vi "CSM - Debug Console 2.vi"() -> ()   [LabVIEW 2017, in "DebugConsole.lvlib"]
doc: "New version of the CSM Debug Console, you can use this tool:\n1. Select an existing CSM instance, open the front panel and block diagram.\n2. Scan the API interfaces of existing CSM instances.\n3. Select an API interface, call synchronously or asynchronously, view the return value.\n4. View the overall program's running log.\n5. Run Scripts."
uses:
  DebugConsole.lvlib
  _Support/Typedef/_CSM_List Module Scope.ctl
  _Support/Typedef/_CSM_GlobalLog_MSG.ctl
  _Support/Typedef/_CSM_Response Source Message.ctl
  _Support/Typedef/_CSM_GlobalLog_MSG_TYPE.ctl
  _BroadcastDef.ctl
  AdvanceAPI/CSM - Convert Error to Argument.vi
  _Support/GlobalEvent/GEvt-Generate with Rule Check.vi
  _Support/GlobalEvent/Cache-GEvt Refs.vi
  AdvanceAPI/CSM - Keywords.vi
  AdvanceAPI/CSM - Make String Arguments Safe.vi
  _Support/ChangeFlag/FlagInstance-GEvt Refs.vi
  _Support/ChangeFlag/ChangeFlag-Read.vi
  _csmHelper/API/Create From VI Reference.vi
  _csmHelper/API/Update lvcsm Section in VI Description.vi
  _csmHelper/API/Destroy.vi
  _csmlite/_PassAllowedMessage - MsgList.vi
  _Support/ChangeFlag/ChangeFlagDB.vi
  _Support/GlobalEvent/FGV-GlobalEventRef(lvlibp).vi
  _Support/GlobalEvent/FGV-GlobalEventQueues(lvlibp).vi
  _Support/GlobalEvent/GEvt-Valid Subscribers.vi
  _Support/GlobalEvent/LogFilter/LogFilter - Check.vi
  HistoryList.vi
  Script-Window.vi
  Module Information.vi
  _Support/GlobalEvent/LogFilter/LogFilter.lvclass
  Communicable State Machine.lvlib
  _csmHelper/API with lvcsm Support/CSM-Helper API with lvcsm Support.lvlib
  _csmHelper/CSM-Helper.lvclass
  _ui/csm-ui-support.lvlib
  _csmlite/_csmlite.lvlib
  _Shared/CSM Shared.lvlib
  _csmlite/_action.ctl
panel:
  in  "Scope":T1
  in  "Refresh CSMs Button":bool
  in  "CSM":string(combo)
  in  "Write lvcsm in Description":bool
  out "inlvlibp":bool
  in  "RetainWireValues":bool
  in  "Toolbar.Exit":bool
  in  "Toolbar.Open FP":bool
  in  "Toolbar.Open BD":bool
  in  "Refresh lvcsm Cache":bool
  in  "Console":T2(tab)
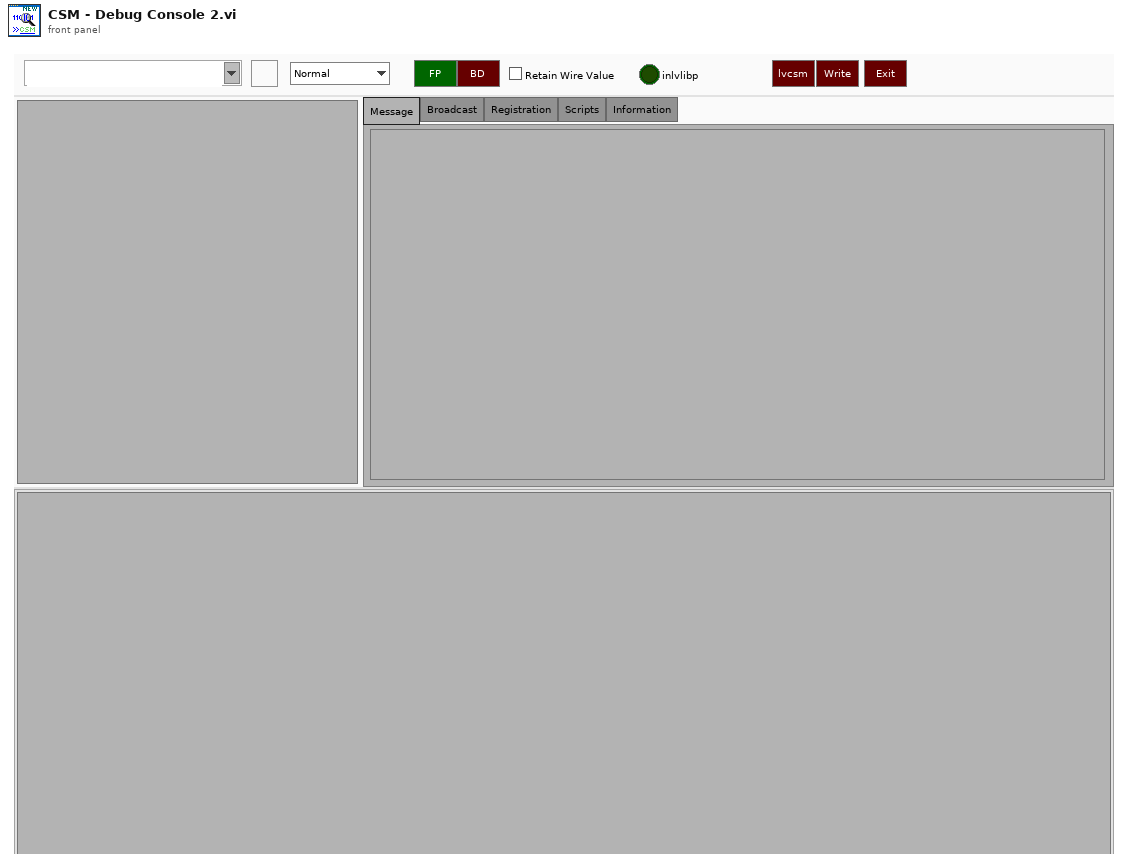
[diagram p1: front panel]
types:
  T1 = typedef "Communicable State Machine.lvlib/_CSM_List Module Scope.ctl" = enum16{"Normal", "System Only", "All"}
  T2 = enum32{"Message", "Broadcast", "Registration", "Scripts", "Information"}
  T3 = cluster{"Left":i32, "Right":i32, "Top":i32, "Bottom":i32}
  T4 = enum32{"Invalid", "Standard", "Closed", "Hidden", "Minimized", "Maximized"}
  T5 = enum32{"invalid app kind", "Development System", "Run Time System", "Student Edition", "Embedded LabVIEW", "Evaluation", "Custom"}
  T6 = typedef "DebugConsole.lvlib/_BroadcastDef.ctl" = enum16{"<no action>", "Macro: Exit", "CSM: Module List Changed", "CSM: Scripts Changed", "CSM: Registration Changed", "CSM: Module Selected", "CSM: Message Excuted", "CSM: Broadcast Excuted", "CSM: Registration Action Excuted", "UI: Try to Change Command"}
  T7 = typedef "_csmlite.lvlib/_action.ctl" = enum16{"Obtain", "Destroy", "Broadcast", "Post", "List"}
  T8 = cluster{"Shift":bool, "Ctrl":bool, "Alt":bool, "Cmd":bool, "Opt":bool}
  T9 = cluster{"Core":cluster{"Current VI Reference":refnum<vi>, "Close Panel on Exit?":bool}, "CSM Global Log Event":refnum<user-event>, "MessageList":string[], "Toobar.advance":refnum<vi>[], "ConsoleUI":refnum<vi>[]}
  T10 = cluster{"Current VI Reference":refnum<vi>, "Close Panel on Exit?":bool}
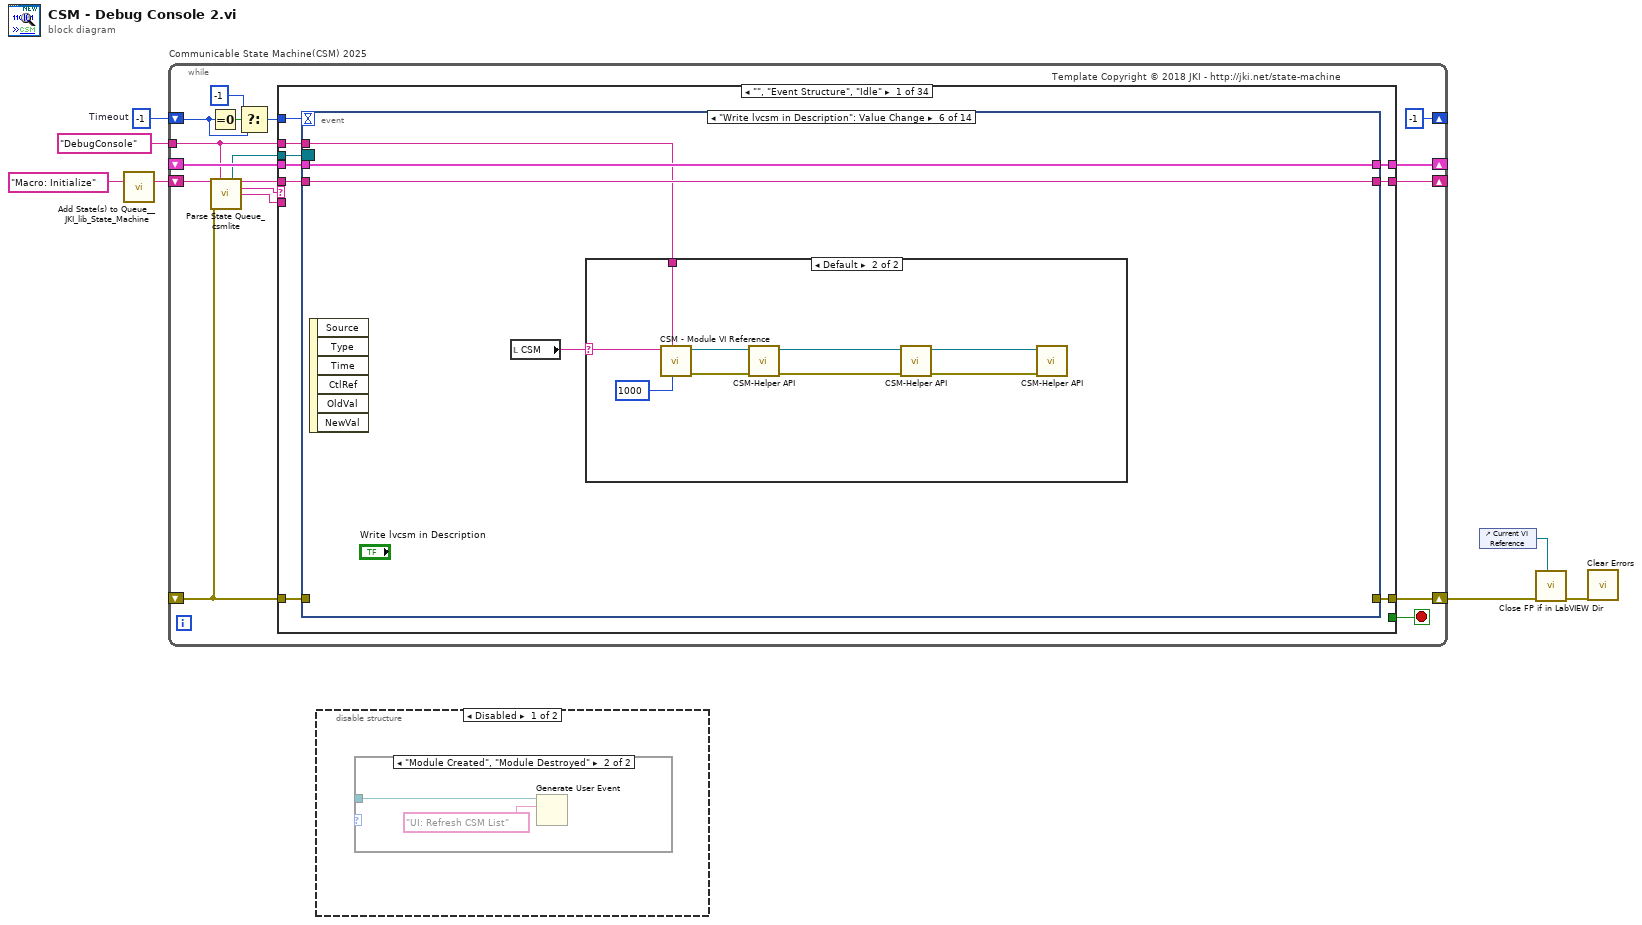
[diagram p0: block diagram]
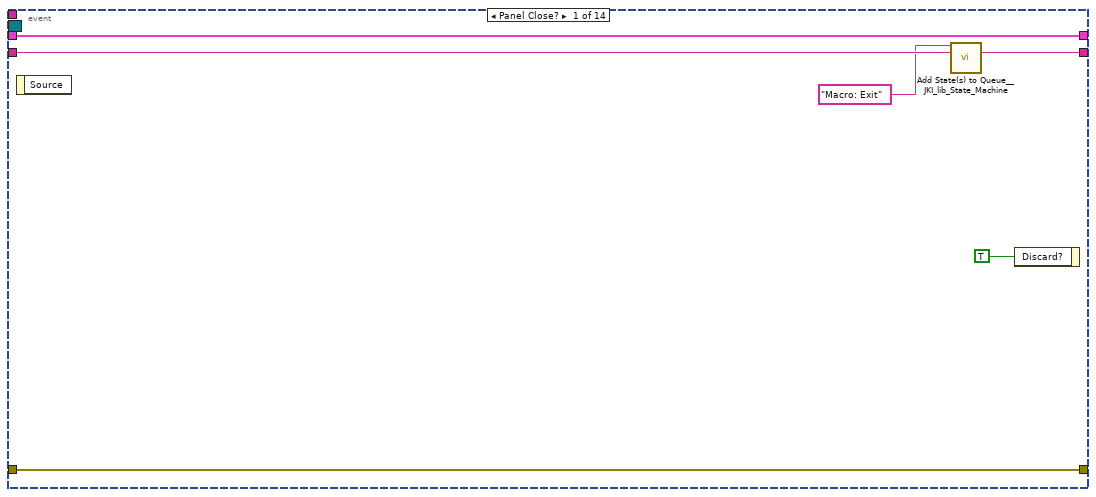
[diagram p4: hidden frame]
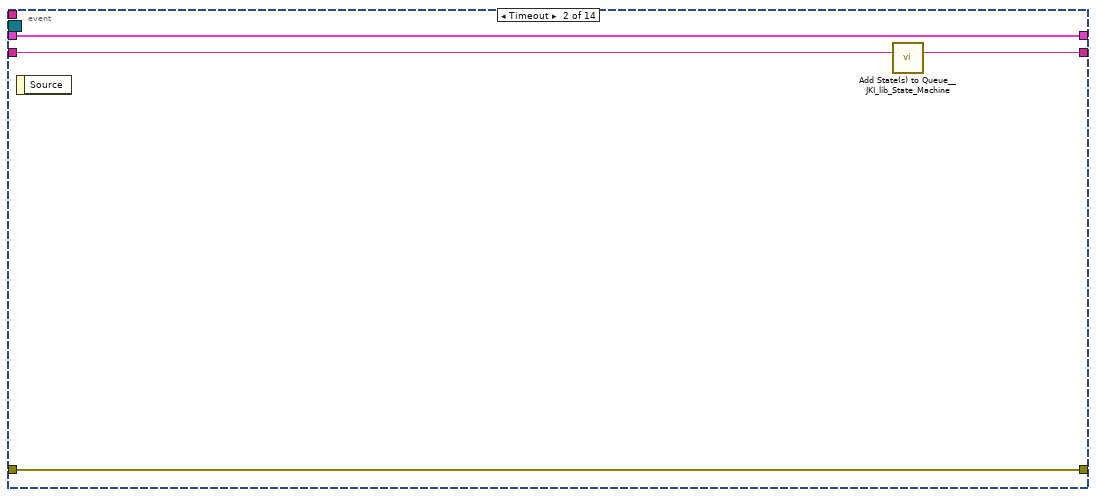
[diagram p5: hidden frame]
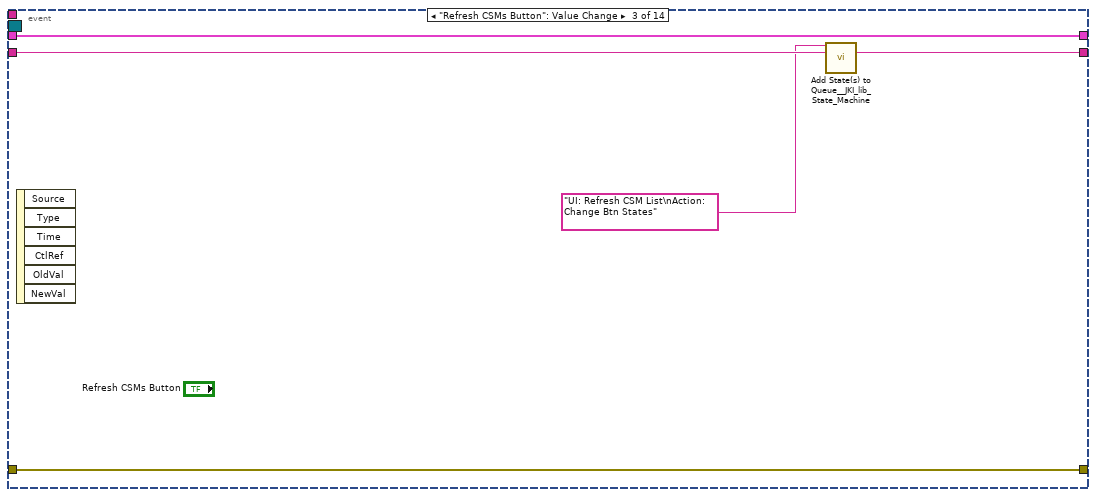
[diagram p6: hidden frame]
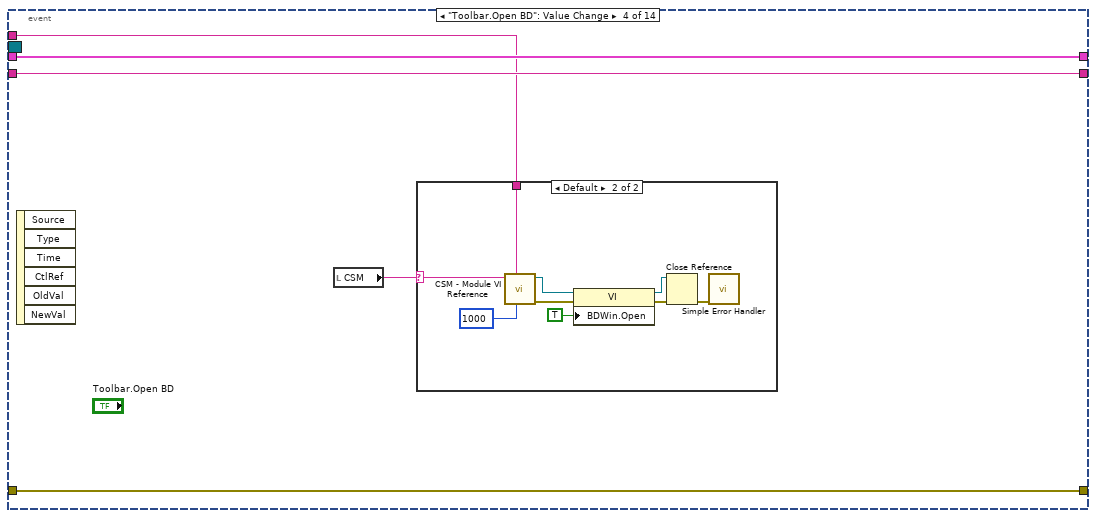
[diagram p7: hidden frame]
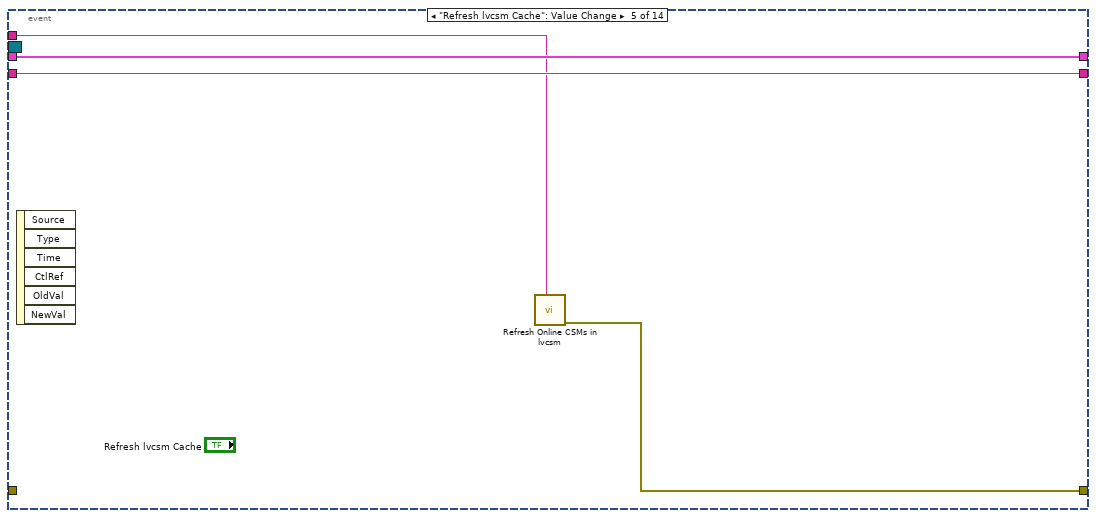
[diagram p9: hidden frame]
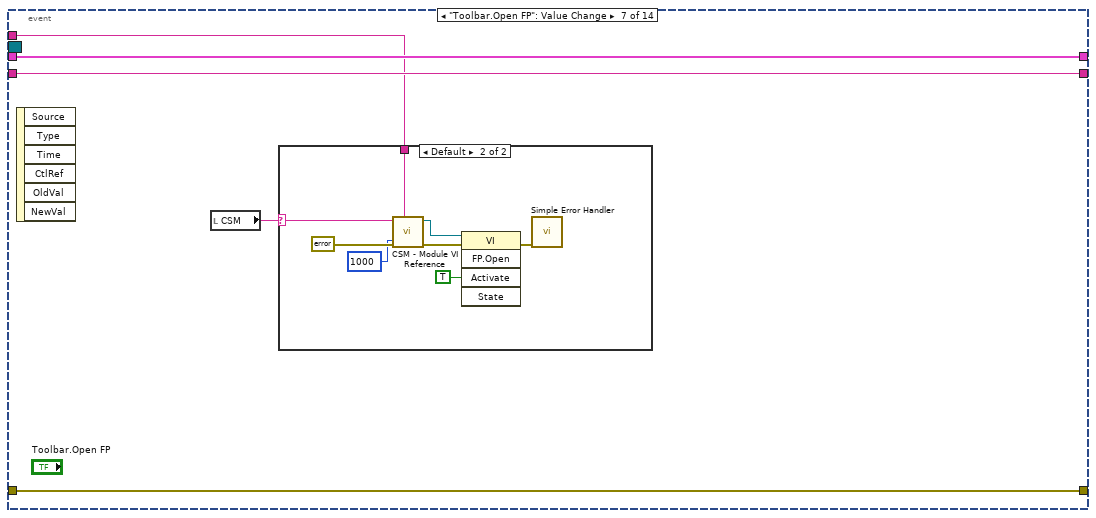
[diagram p11: hidden frame]
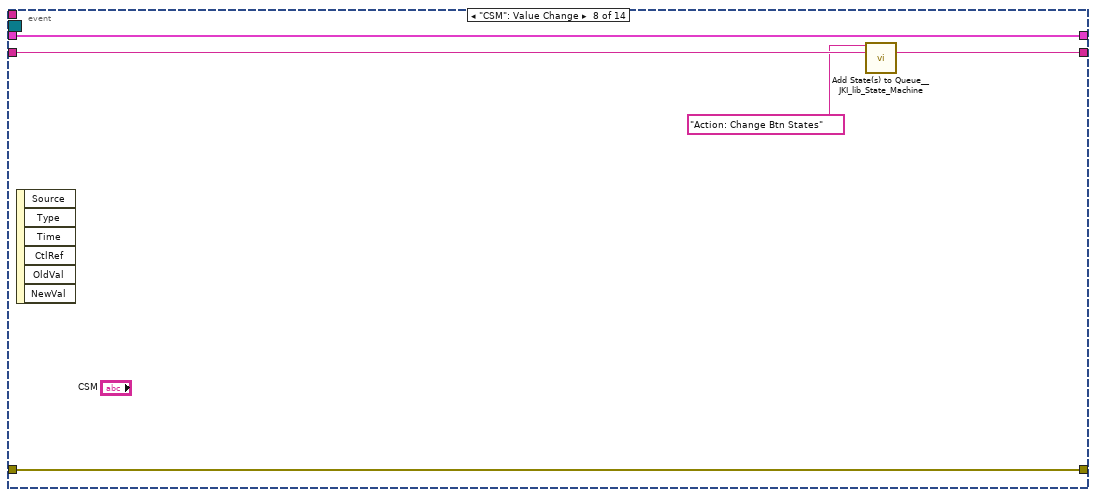
[diagram p13: hidden frame]
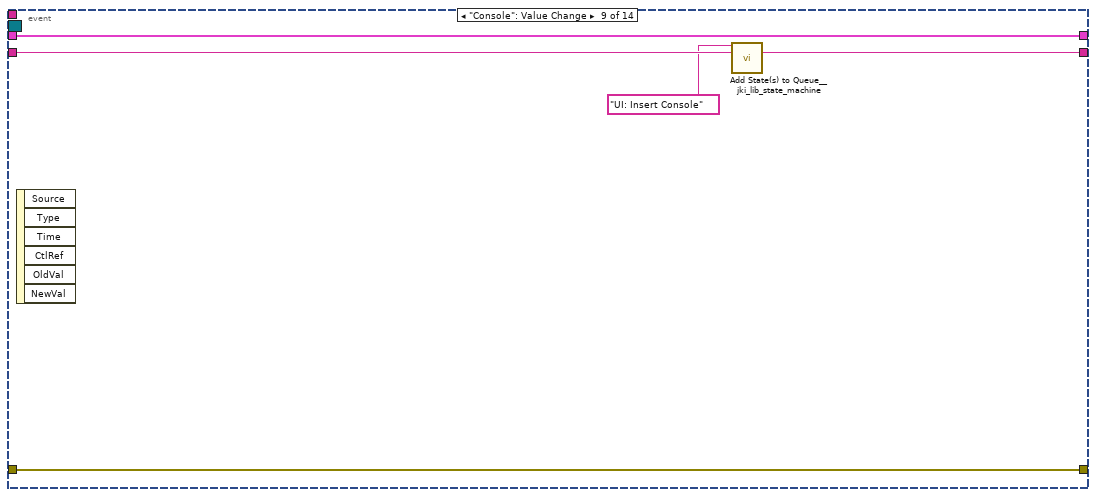
[diagram p14: hidden frame]
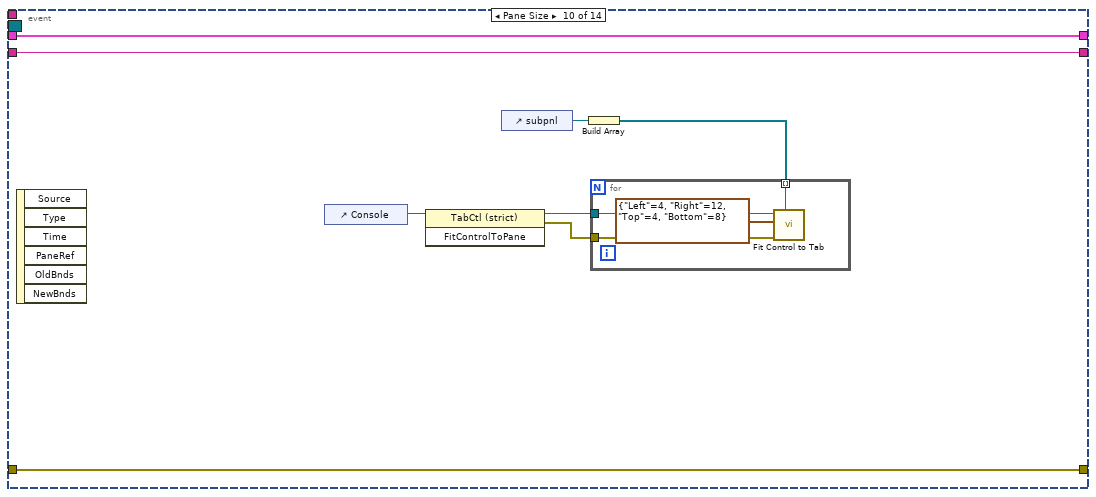
[diagram p15: hidden frame]
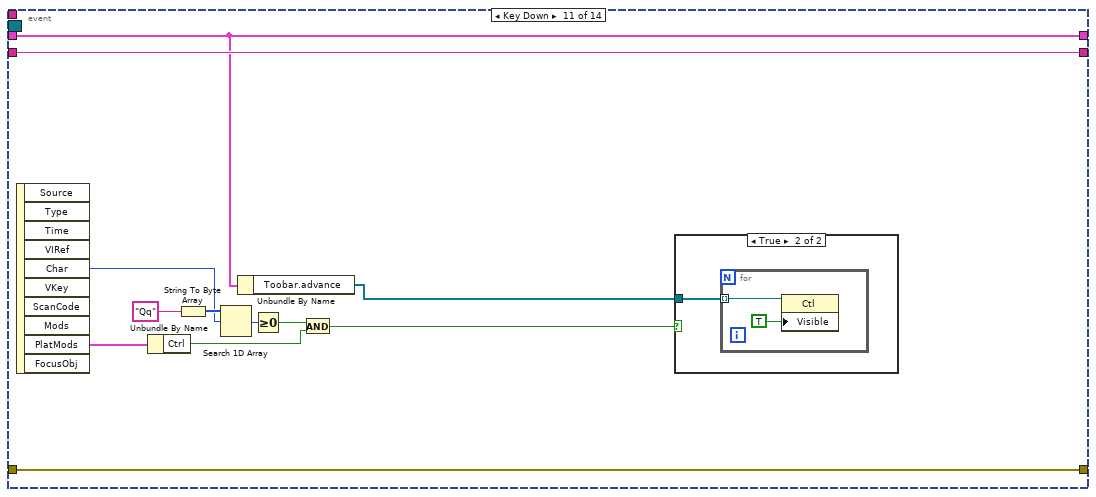
[diagram p16: hidden frame]
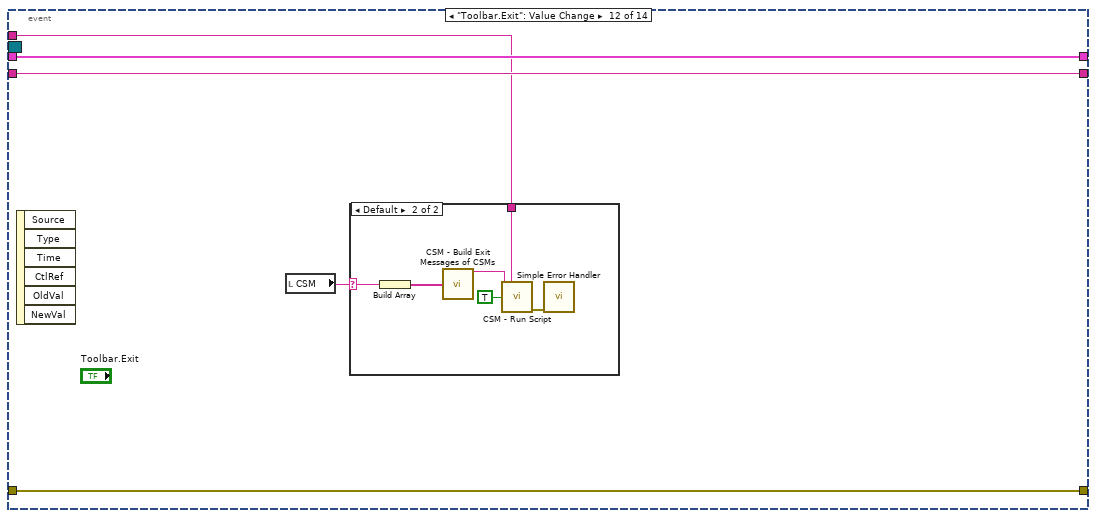
[diagram p18: hidden frame]
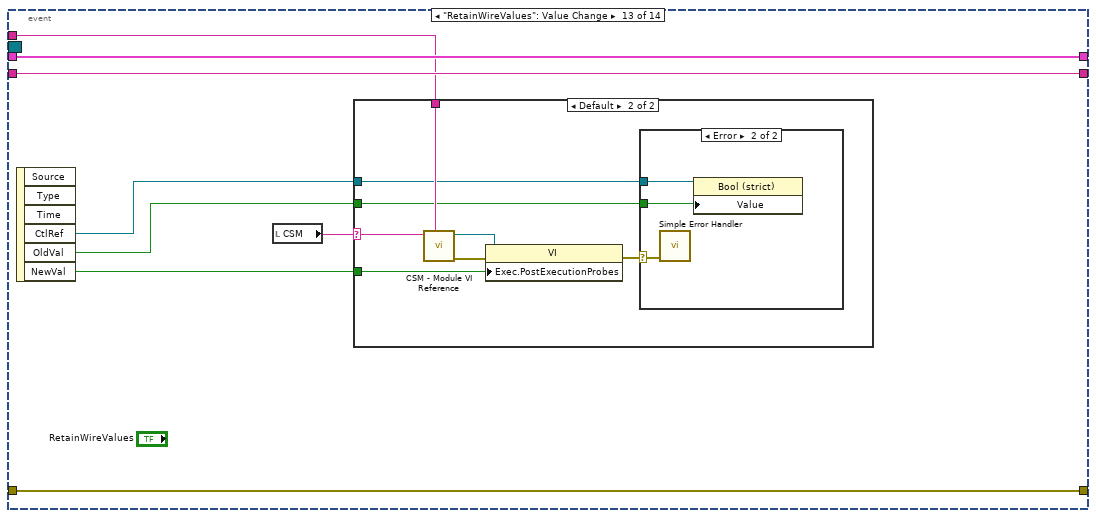
[diagram p20: hidden frame]
diagram:
  w5 = -1  # Timeout
  n1 = call <vilib>:"Add State(s) to Queue__JKI_lib_State_Machine.vi"("State(s) in (\"\")"="Macro: Initialize") -> ("States Out"=w6:string)  [unwired: 14 in]
  n2 = while "Communicable State Machine(CSM) 2025" {
    shift-right: [w17] -> _
    shift-left: _ -> [w16]
    shift-right: [w20] -> w2
    shift-left: _ -> [w15]
    shift-right: [w19] -> _
    shift-left: w6 -> [w21]
    tunnel: "DebugConsole" -> [w9]
    shift-right: [-1 ("Timeout")] -> _
    shift-left: w5 -> [w12]
    stop <- w18 stop-if-true
    # "Template Copyright © 2018 JKI - http://jki.net/state-machine"
    n3 = Equal To 0?(x=w12) -> (x = 0?=w14:bool)
    n4 = call "Parse State Queue_csmlite.vi"("State Queue"=w21, "Current Module(\"\" to generate an ID)"=w9, "Error In (no error)"=w15) -> ("Event Registration Refnum"=w8:refnum<event-registration>, "Remaining States"=w23:string, "Current State"=w24:string, "Arguments"=w22:string)  [unwired: 9 in]
    n5 = Select(t=-1 ("Timeout"), s=w14, f=w12) -> (s? t:f=w11:i32)
    n6 = case shown="\"\", \"Event Structure\", \"Idle\"" w24 {
      selector: w24 -> [_ _ w171 _ _ _ _ _ _ _ _ _ _ _ _ _ _ _ _ _ _ _ _ _ _ _ _ _ _ _ _ _ _ _]
      tunnel: w23 -> [w33 w170 w175 w194 w201 w206 w210 w219 w226 w229 w231 w241 w256 w260 w270 w280 w291 w368 w385 w405 w421 w428 w431 w436 w441 w452 w473 w479 w498 w503 w522 w541 w560 w579]
      tunnel: w22 -> [_ _ _ _ _ _ _ _ _ _ _ w237 _ _ _ w275 w285 _ w382 _ _ _ _ _ _ _ _ _ _ _ _ _ _ _]
      tunnel: w16 -> [w31 w167 w173 w187 w198 w204 w207 _ w225 w228 w230 w239 w251 w257 w267 w278 w287 w367 w384 w404 w420 w426 w430 w433 w438 w449 w470 w478 w497 w502 w521 w540 w559 w578]
      tunnel: [w30 w168 w177 w191 errorcluster {"status"=FALSE, "code"=0, "source"=""} ("error out") w203 w208 w216 w227 _ _ w240 w252 w258 w268 w276 w288 w369 w386 w406 w422 w429 w432 w434 w439 w450 w471 w480 w499 w504 w523 w542 w561 w580] -> w20
      tunnel: w15 -> [w29 w168 w176 w191 w197 w203 w208 w216 w227 _ _ w240 w253 w258 w268 w277 w289 w369 w386 w406 w422 w429 w432 w434 w439 w450 w471 w480 w499 w504 w523 w542 w561 w580]
      tunnel: [w32 w169 w174 w193 w200 w205 w209 w218 w226 w229 w231 w241 w255 w259 w269 w279 w290 w368 w385 w405 w421 w428 w431 w435 w440 w451 w472 w479 w498 w503 w522 w541 w560 w579] -> w19
      tunnel: [_ _ _ _ _ TRUE _ _ _ _ _ _ _ _ _ _ _ _ _ _ _ _ _ _ _ _ _ _ _ _ _ _ _ _] -> w18
      tunnel: [w28 w167 w173 w192 w198 w204 w207 w217 w222 w228 w230 w233 w251 w257 w267 w278 w287 w367 w384 w404 w420 w426 w430 w433 w438 w449 w470 w478 w497 w501 w520 w539 w558 w577] -> w17
      tunnel: w11 -> [w27 _ _ _ _ _ _ _ _ _ _ _ _ _ _ _ _ _ _ _ _ _ _ _ _ _ _ _ _ _ _ _ _ _]
      tunnel: w9 -> [w26 _ _ _ w195 _ _ _ _ _ _ _ _ _ _ _ _ _ _ w393 w409 _ _ _ _ w442 _ w476 w495 w500 w519 w538 w557 w576]
      tunnel: w8 -> [w25 _ _ _ _ _ _ _ _ _ _ _ _ _ _ _ _ _ _ _ _ _ _ _ _ _ _ _ _ _ _ _ _ _]
      frame "", "Event Structure", "Idle" {
        n7 = event shown="[5] \"Write lvcsm in Description\": Value Change" {
          selector: w25 -> [_ _ _ _ _ _ _ _ _ _ _ _ _ _]
          dyn-events: _ -> [_ _ _ _ _ _ _ _ _ _ _ _ _ _]
          timeout: w27 -> [_ _ _ _ _ _ _ _ _ _ _ _ _ _]
          tunnel: w33 -> [w39 w43 w46 w53 w66 w70 w84 w94 w99 w110 w126 w134 w148 w163]
          tunnel: [w38 w42 w45 w53 w66 w70 w84 w95 w100 w110 w126 w134 w148 w164] -> w32
          tunnel: w31 -> [w36 w40 w47 w52 w65 w69 w83 w96 w101 w108 w115 w133 w146 w165]
          tunnel: [w37 w41 w48 w50 w63 _ w81 w97 w102 w109 w125 w132 w147 w166] -> w30
          tunnel: w29 -> [w37 w41 w48 w50 _ _ w81 w97 w102 w109 w125 w132 w147 w166]
          tunnel: [w36 w40 w47 w52 w65 w69 w83 w96 w101 w108 w115 w133 w146 w165] -> w28
          tunnel: w26 -> [_ _ _ w49 w64 w67 w80 _ _ _ _ w130 w144 _]
          event Panel Close? {
            n8 = event-data() -> ()  [unwired: 1 in, 1 out]
            n9 = call <vilib>:"Add State(s) to Queue__JKI_lib_State_Machine.vi"("State(s) in Front (\"\")"="Macro: Exit", "State(s) in (\"\")"=w39) -> ("States Out"=w38:string)  [unwired: 13 in]
            n10 = event-data("Discard?"=TRUE) -> ()  [unwired: 1 in, 1 out]
          }
          event Timeout {
            n11 = event-data() -> ()  [unwired: 1 in, 1 out]
            n12 = call <vilib>:"Add State(s) to Queue__JKI_lib_State_Machine.vi"("State(s) in (\"\")"=w43) -> ("States Out"=w42:string)  [unwired: 14 in]
          }
          event "Refresh CSMs Button": Value Change {
            n13 = event-data() -> ()  [unwired: 1 in, 6 out]
            n14 = call <vilib>:"Add State(s) to Queue__JKI_lib_State_Machine.vi"("State(s) in Front (\"\")"="UI: Refresh CSM List\nAction: Change Btn States" ("State(s) in Front (\"\")"), "State(s) in (\"\")"=w46) -> ("States Out"=w45:string)  [unwired: 13 in]
          }
          event "Toolbar.Open BD": Value Change {
            n15 = event-data() -> ()  [unwired: 1 in, 6 out]
            n16 = local read "CSM"() -> (w51:string)
            n17 = case shown="Default" w51 {
              selector: w51 -> [_ w61]
              tunnel: w49 -> [_ w60]
              frame "" {
              }
              frame Default {
                n18 = call "CSM - Module VI Reference.vi"("Response Timeout (-2 Using Global Settings)"=1000 ("Response Timeout(5000 ms)"), "Current Module (\"\" to Generate an ID)"=w60, "CSM Name"=w61) -> ("error out"=w54:errorcluster, "CSM Module VIRef"=w59:refnum<vi>)  [unwired: 7 in]
                n19 = property class="VI"(reference=w59, error in=w54, "BDWin.Open"=TRUE ("Block Diagram Window:Open")) -> (reference out=w57:refnum<vi>, error out=w56:errorcluster)
                n20 = Close Reference(reference=w57, error in (no error)=w56) -> (error out=w62:errorcluster)
                n21 = call <vilib>:"Simple Error Handler.vi"("error in (no error)"=w62) -> ()  [unwired: 4 in, 5 out]
              }
            }
          }
          event "Refresh lvcsm Cache": Value Change {
            n22 = event-data() -> ()  [unwired: 1 in, 6 out]
            n23 = call "Refresh Online CSMs in lvcsm.vi"("Caller"=w64) -> ("error out"=w63:errorcluster)  [unwired: 9 in, 1 out]
          }
          event "Write lvcsm in Description": Value Change {
            n24 = event-data() -> ()  [unwired: 1 in, 6 out]
            n25 = local read "CSM"() -> (w68:string)
            n26 = case shown="Default" w68 {
              selector: w68 -> [_ w75]
              tunnel: w67 -> [_ w71]
              frame "" {
              }
              frame Default {
                n27 = call "CSM - Module VI Reference.vi"("Response Timeout (-2 Using Global Settings)"=1000 ("Response Timeout(5000 ms)"), "Current Module (\"\" to Generate an ID)"=w71, "CSM Name"=w75) -> ("error out"=w73:errorcluster, "CSM Module VIRef"=w72:refnum<vi>)  [unwired: 7 in]
                n28 = call-poly "CSM-Helper API.vi"("error in (no error)"=w73, "VI"=w72) -> ("error out"=w79:errorcluster, "CSM-Helper.lvclass"=w78:refnum<class "CSM-Helper.lvclass">)  [unwired: 8 in]
                n29 = call-poly "CSM-Helper API.vi"("error in (no error)"=w79, "CSM-Helper in"=w78) -> ("error out"=w77:errorcluster, "CSM-Helper out"=w76:refnum<class "CSM-Helper.lvclass">)  [unwired: 8 in]
                n30 = call-poly "CSM-Helper API.vi"("error in (no error)"=w77, "CSM-Helper in"=w76) -> ()  [unwired: 8 in, 2 out]
              }
            }
          }
          event "Toolbar.Open FP": Value Change {
            n31 = event-data() -> ()  [unwired: 1 in, 6 out]
            n32 = local read "CSM"() -> (w82:string)
            n33 = case shown="Default" w82 {
              selector: w82 -> [_ w92]
              tunnel: w80 -> [_ w90]
              frame "" {
              }
              frame Default {
                n34 = call "CSM - Module VI Reference.vi"("Response Timeout (-2 Using Global Settings)"=1000 ("Response Timeout(5000 ms)"), "Current Module (\"\" to Generate an ID)"=w90, "error in (no error)"=errorcluster {"status"=FALSE, "code"=0, "source"=""}, "CSM Name"=w92) -> ("error out"=w86:errorcluster, "CSM Module VIRef"=w87:refnum<vi>)  [unwired: 6 in]
                n35 = invoke on="Invoke Node" class="VI" method="FP.Open"(reference=w87, error in=w86, "Activate"=TRUE ("Activate?")) -> (error out=w91:errorcluster)  [unwired: 2 in, 4 out]
                n36 = call <vilib>:"Simple Error Handler.vi"("error in (no error)"=w91) -> ()  [unwired: 4 in, 5 out]
              }
            }
          }
          event "CSM": Value Change {
            n37 = event-data() -> ()  [unwired: 1 in, 6 out]
            n38 = call <vilib>:"Add State(s) to Queue__JKI_lib_State_Machine.vi"("State(s) in Front (\"\")"="Action: Change Btn States" ("State(s) in Front (\"\")"), "State(s) in (\"\")"=w94) -> ("States Out"=w95:string)  [unwired: 13 in]
          }
          event "Console": Value Change {
            n39 = event-data() -> ()  [unwired: 1 in, 6 out]
            n40 = call <vilib>:"Add State(s) to Queue__jki_lib_state_machine.vi"("State(s) in Front (\"\")"="UI: Insert Console" ("State(s) in Front (\"\")"), "State(s) in (\"\")"=w99) -> ("States Out"=w100:string)  [unwired: 13 in]
          }
          event Pane Size {
            n41 = event-data() -> ()  [unwired: 1 in, 6 out]
            n42 = control-ref of="Console"() -> (w105:refnum<vi>)
            n43 = invoke class="TabCtl (strict)" method="FitControlToPane"(reference=w105) -> (reference out=w107:refnum<vi>, error out=w106:errorcluster)  [unwired: 2 in, 1 out]
            n44 = control-ref of="subpnl"() -> (w104:refnum<vi>)
            n45 = Build Array(w104) -> (w103:refnum<vi>[])
            n46 = for {
              tunnel: w107 -> [w114]
              tunnel: w103 -> [w113] mode=indexing
              tunnel: w106 -> [w112]
              n47 = call "Fit Control to Tab.vi"("Control"=w113, "error in (no error)"=w112, "Margin"=T3 {"Left"=4, "Right"=12, "Top"=4, "Bottom"=8}, "TabRef"=w114) -> ()  [unwired: 3 in, 3 out]
            }
          }
          event Key Down {
            n48 = event-data() -> ("Char"=w116:i16, "PlatMods"=w117:T8)  [unwired: 1 in, 8 out]
            n49 = Unbundle By Name(w117) -> ("Ctrl"=w120:bool)
            n50 = String To Byte Array(string="Qq") -> (unsigned byte array=w122:u8[])
            n51 = Search 1D Array(1D array=w122, element=w116) -> (index of element=w123:i32)  [unwired: 1 in]
            n52 = Unbundle By Name(w115) -> ("Toobar.advance"=w118:refnum<vi>[])
            n53 = Greater Or Equal To 0?(x=w123) -> (x >= 0?=w124:bool)
            n54 = And(x=w124, y=w120) -> (x .and. y?=w119:bool)
            n55 = case shown="True" w119 {
              tunnel: w118 -> [_ w127]
              frame False {
              }
              frame True {
                n56 = for {
                  tunnel: w127 -> [w129] mode=indexing
                  n57 = property class="Ctl"(reference=w129, "Visible"=TRUE) -> ()  [unwired: 1 in, 2 out]
                }
              }
            }
          }
          event "Toolbar.Exit": Value Change {
            n58 = event-data() -> ()  [unwired: 1 in, 6 out]
            n59 = local read "CSM"() -> (w131:string)
            n60 = case shown="Default" w131 {
              selector: w131 -> [_ w137]
              tunnel: w130 -> [_ w140]
              frame "" {
              }
              frame Default {
                n61 = Build Array(w137) -> (w136:string[])
                n62 = call "CSM - Build Exit Messages of CSMs.vi"("CSMs"=w136) -> ("States"=w138:string)  [unwired: 14 in]
                n63 = call "CSM - Run Script.vi"("CSM Scripts"=w138, "Current Module (\"\" to Generate an ID)"=w140, "Continue If Error? (F)"=TRUE) -> ("error out"=w139:errorcluster)  [unwired: 10 in, 2 out]
                n64 = call <vilib>:"Simple Error Handler.vi"("error in (no error)"=w139) -> ()  [unwired: 4 in, 5 out]
              }
            }
          }
          event "RetainWireValues": Value Change {
            n65 = event-data() -> ("CtlRef"=w142:refnum<vi>, "OldVal"=w141:bool, "NewVal"=w143:bool)  [unwired: 1 in, 3 out]
            n66 = local read "CSM"() -> (w145:string)
            n67 = case shown="Default" w145 {
              selector: w145 -> [_ w154]
              tunnel: w144 -> [_ w153]
              tunnel: w143 -> [_ w152]
              tunnel: w142 -> [_ w150]
              tunnel: w141 -> [_ w149]
              frame "" {
              }
              frame Default {
                n68 = call "CSM - Module VI Reference.vi"("Current Module (\"\" to Generate an ID)"=w153, "CSM Name"=w154) -> ("error out"=w156:errorcluster, "CSM Module VIRef"=w155:refnum<vi>)  [unwired: 8 in]
                n69 = property class="VI"(reference=w155, error in=w156, "Exec.PostExecutionProbes"=w152) -> (error out=w151:errorcluster)  [unwired: 1 out]
                n70 = case shown="Error" w151 {
                  selector: w151 -> [_ w157]
                  tunnel: w150 -> [_ w159]
                  tunnel: w149 -> [_ w158]
                  frame No Error {
                  }
                  frame Error {
                    n71 = call <vilib>:"Simple Error Handler.vi"("error in (no error)"=w157) -> ()  [unwired: 4 in, 5 out]
                    n72 = property class="Bool (strict)"(reference=w159, "Value"=w158) -> ()  [unwired: 1 in, 2 out]
                  }
                }
              }
            }
          }
          event User Event {
            n73 = event-data() -> ("Message Event"=w162:string)  [unwired: 1 in]
            n74 = call-poly "Pass Allowed Message.vi"("Allowed Message"=string[] ["Macro: Exit", "CSM: Module List Changed", "UI: Try to Change Command"], "JKISM External Event"=w162) -> ("States"=w161:string)  [unwired: 7 in]
            n75 = call <vilib>:"Add State(s) to Queue__JKI_lib_State_Machine.vi"("State(s) in Front (\"\")"=w161, "State(s) in (\"\")"=w163) -> ("States Out"=w164:string)  [unwired: 13 in]
          }
        }
      }
      frame "---------- Core ----------" {
        # "Do not put any code in this frame.\n(it is a separator no-op)"
        n76 = call <vilib>:"Add State(s) to Queue__JKI_lib_State_Machine.vi"("State(s) in (\"\")"=w170) -> ("States Out"=w169:string)  [unwired: 14 in]
      }
      frame Default {
        w180 = 42 items=["No error", "Argument error", "Memory is full", "Out of zone", "End of file", "File already open", "Generic file I/O error", "File not found", "File permission error", "Disk is full", "Duplicate path", "Too many files open", "System feature not enabled", "Resource file not found", "Cannot add resource", "Resource not found", "Image not found", "Image memory error", "Pen does not exist", "Config type invalid", "Config token not found", "Config parse error", "Config memory error", "Bad external code format", "Bad external code offset", "External code not present", "Null window", "Destroy window error", "Null menu", "Print aborted", "Bad print record", "Print driver error", "Windows error during printing", "Memory error during printing", "Print dialog error", "Generic print error", "Invalid device refnum", "Device not found", "Device parameter error", "Device unit error", "Cannot open device", "Device call aborted", "Generic error", "Cancelled by user", "Object ID too low", "Object ID too high", "Object not in heap", "Unknown heap", "Unknown object (invalid DefProc)", "Unknown object (DefProc not in table)", "Message out of range", "Invalid (null) method", "Unknown message", "Manager call not supported", "Bad address", "Network operation in progress", "Network operation timed out", "Connection is busy", "Network attribute not supported", "Network error", "Address in use", "System out of memory", "Connection aborted", "Connection refused", "Not connected", "Already connected", "Connection closed", "Initialization error (interapplication manager)", "Bad occurrence", "Wait on unbound occurrence handler", "Occurrence queue overflow", "Datalog type conflict", "Unused", "Unrecognized type (interapplication manager)", "Memory corrupt", "Failed to make temporary DLL", "Old CIN version", "Drag socket not found", "Failed to load drop-object", "Failed to register OLE object", "Failed to release OLE object", "Format specifier type mismatch", "Unknown format specifier", "Too few format specifiers", "Too many format specifiers", "Scan failed", "Newer CIN version", "Error converting to variant", "Runtime menu error", "Password tampered", "Variant attribute not found", "Incompatible variant data type", "Event data is not available", "Event Store is not present", "Occurrence is not found", "Event Queue is not created", "Event info is not available", "Refnum passed is NULL", "Error retrieving Class GUID", "Error retrieving CoClass GUID", "Error retrieving TypeLib GUID.", "Bad built application magic bytes.", "Specific driver is different from the specific driver associated with the Logical Name.", "There is no session opened to the class driver.", "Max Error", "MAX - Error with config objects", "MAX - Error loading configuration", "MAX - Group not supported"]
        # "Current State"
        # "Do not delete, rename, or modify this frame.\n(this is used to capture unhandled states and typos)"
        # "Handle mistyped state name (developer tool)"
        n77 = Format Into String(format string="Software Exception: Unhandled State \"%s\"." ("message"), error in=w176, w171) -> (resulting string=w179:string, error out=w178:errorcluster)  [unwired: 1 in]
        n78 = call <vilib>:"Error Cluster From Error Code.vi"("show call chain? (False)"=TRUE, "error in (no error)"=w178, "error message (\"\")"=w179, "error code (0)"=w180) -> ("error out"=w177:errorcluster)  [unwired: 5 in]
        n79 = call <vilib>:"Add State(s) to Queue__JKI_lib_State_Machine.vi"("State(s) in (\"\")"=w175) -> ("States Out"=w174:string)  [unwired: 14 in]
      }
      frame "Initialize Core Data" {
        # "Do not delete, rename, or modify this frame.\n(this is used to determine panel behavior on exit)"
        # "originally closed?"
        # "exe?"
        # "If panel starts closed or is an EXE, then close it when we exit"
        n80 = property class="VI"() -> ("FP.State"=w184:T4)  [unwired: 2 in, 2 out]
        n81 = property class="App"() -> ("App.Kind"=w190:T5)  [unwired: 2 in, 2 out]
        n82 = control-ref of="Current VI Reference"() -> (w185:refnum<vi>)
        n83 = Equal?(x=w184, y=T4."Closed" ("Front Panel Window:State")) -> (x = y?=w182:bool)
        n84 = Equal?(x=w190, y=T5."Run Time System" ("Application:Kind")) -> (x = y?=w188:bool)
        n85 = Or(x=w182, y=w188) -> (x .or. y?=w186:bool)
        n86 = Bundle By Name(cluster=w187, "Core.Current VI Reference"=w185, "Core.Close Panel on Exit?"=w186) -> (w192:T9)
        n87 = call <vilib>:"Add State(s) to Queue__JKI_lib_State_Machine.vi"("State(s) in (\"\")"=w194) -> ("States Out"=w193:string)  [unwired: 14 in]
      }
      frame "Error Handler" {
        # "Unhandled Error -- Display it"
        # "Handle any errors here.\nYou can also output any states to clean-up after errors occur"
        # "Clear error"
        n88 = call "CSM - Global Log Error Handler.vi"("Place (\"\" to Use VI's Name)"=w195, "Error In"=w197) -> ()  [unwired: 9 in, 1 out]
        n89 = call <vilib>:"Add State(s) to Queue__JKI_lib_State_Machine.vi"("State(s) in Front (\"\")"="/* Post Error States", "State(s) in (\"\")"=w201) -> ("States Out"=w200:string)  [unwired: 13 in]
      }
      frame "Exit" {
        # "Do not put any code in this frame.\n(No errors that occur here will be handled.)"
        n90 = call <vilib>:"Add State(s) to Queue__JKI_lib_State_Machine.vi"("State(s) in (\"\")"=w206) -> ("States Out"=w205:string)  [unwired: 14 in]
      }
      frame "---------- Data ----------" {
        # "Do not put any code in this frame.\n(It is a separator no-op. You can make a copy of this frame to create a new Data frame)"
        n91 = call <vilib>:"Add State(s) to Queue__JKI_lib_State_Machine.vi"("State(s) in (\"\")"=w210) -> ("States Out"=w209:string)  [unwired: 14 in]
      }
      frame "Data: Initialize" {
        w211 = refnum<vi>[] []  # ConsoleUI
        w212 = refnum<vi>[] []  # Toobar.advance
        w213 = string[] []  # MessageList
        w214 = refnum<user-event> refnum  # CSM Global Log Event
        w215 = T10 {"Current VI Reference"=refnum, "Close Panel on Exit?"=FALSE}  # Core
        # "Initialize the shift-register data, here.\n(data names are defined by what you wire into the bundle function)"
        n92 = Bundle("Core"=w215, "CSM Global Log Event"=w214, "MessageList"=w213, "Toobar.advance"=w212, "ConsoleUI"=w211) -> (w217:T9)  [unwired: 1 in]
        n93 = call <vilib>:"Add State(s) to Queue__JKI_lib_State_Machine.vi"("State(s) in (\"\")"=w219) -> ("States Out"=w218:string)  [unwired: 14 in]
      }
      frame "Data: Initialize References" {
        n94 = control-ref of="Toolbar.Open FP"() -> (w224:refnum<vi>)
        n95 = control-ref of="Toolbar.Open BD"() -> (w223:refnum<vi>)
        n96 = control-ref of="Refresh lvcsm Cache"() -> (w220:refnum<vi>)
        n97 = Build Array(w224, w223, w220) -> (w221:refnum<vi>[])
        n98 = Bundle By Name(cluster=w225, "Toobar.advance"=w221) -> (w222:T9)
      }
      frame "Data: Load Arguments Config File" {
      }
      frame "Data: Save Arguments Config File" {
      }
      frame "Data: Update Message List" {
        n99 = Unbundle By Name(w239) -> ("MessageList"=w238:string[])
        n100 = call "CSM - Revert Arguments-Safe String.vi"("Safe Argument String"=w237) -> ("Origin Argument String"=w236:string)  [unwired: 8 in]
        n101 = Build Array (concatenate)(w236, w238) -> (w235:string[])
        n102 = for {
          tunnel: w235 -> [w245] mode=indexing
          shift-right: [w244] -> w232
          shift-left: string[] [] -> [w243]
          i -> [w242]
          n103 = Search 1D Array(1D array=w243, element=w245) -> (index of element=w246:i32)  [unwired: 1 in]
          n104 = case shown="-1" w246 {
            tunnel: w245 -> [_ w250]
            tunnel: [w247 w248] -> w244
            tunnel: w243 -> [w247 w249]
            tunnel: w242 -> [_ _]
            frame Default {
            }
            frame -1 {
              n105 = Build Array (concatenate)(w249, w250) -> (w248:string[])
            }
          }
        }
        n106 = Bundle By Name(cluster=w239, "MessageList"=w232) -> (w233:T9)
      }
      frame "Data: Cleanup" {
        # "Cleanup any data and references, here.\n(this is called automatically, by the Macro: Exit)"
        n107 = Unbundle By Name(w251) -> ("Core.Current VI Reference"=w254:refnum<vi>)
        n108 = Close Reference(reference=w254, error in (no error)=w253) -> (error out=w252:errorcluster)
        n109 = call <vilib>:"Add State(s) to Queue__JKI_lib_State_Machine.vi"("State(s) in (\"\")"=w256) -> ("States Out"=w255:string)  [unwired: 14 in]
      }
      frame "---------- UI ----------" {
        # "Do not put any code in this frame.\n(It is a separator no-op. You can make a copy of this frame to create a new UI frame)"
        n110 = call <vilib>:"Add State(s) to Queue__JKI_lib_State_Machine.vi"("State(s) in (\"\")"=w260) -> ("States Out"=w259:string)  [unwired: 14 in]
      }
      frame "UI: Initialize" {
        # "Initialize the User Interface, here.\n(this is called automatically, by the Macro: Init)"
        n111 = control-ref of="Console"() -> (w264:refnum<vi>)
        n112 = invoke class="TabCtl (strict)" method="FitControlToPane"(reference=w264) -> (reference out=w266:refnum<vi>, error out=w265:errorcluster)  [unwired: 2 in, 1 out]
        n113 = control-ref of="subpnl"() -> (w263:refnum<vi>)
        n114 = local write "Console"(0) -> ()
        n115 = Build Array(w263) -> (w262:refnum<vi>[])
        n116 = for {
          tunnel: w266 -> [w274]
          tunnel: w262 -> [w273] mode=indexing
          tunnel: w265 -> [w272]
          n117 = call "Fit Control to Tab.vi"("Control"=w273, "error in (no error)"=w272, "Margin"=T3 {"Left"=4, "Right"=12, "Top"=4, "Bottom"=8}, "TabRef"=w274) -> ()  [unwired: 3 in, 3 out]
        }
        n118 = call <vilib>:"Add State(s) to Queue__JKI_lib_State_Machine.vi"("State(s) in (\"\")"=w270) -> ("States Out"=w269:string)  [unwired: 14 in]
      }
      frame "UI: Cursor Set" {
        # "Argument"
        # "Set and Unset Cursor Busy.\n(Usage: \"UI: Cursor Set >> Busy|Idle\")"
        n119 = case shown="\"Idle\", Default" w275 {
          tunnel: w277 -> [w282 w284]
          tunnel: [w281 w283] -> w276
          frame "Idle", Default {
            n120 = call <vilib>:"Unset Busy.vi"("error in (no error)"=w282) -> ("error out"=w281:errorcluster)  [unwired: 10 in]
          }
          frame "Busy" {
            n121 = call <vilib>:"Set Busy.vi"("error in (no error)"=w284) -> ("error out"=w283:errorcluster)  [unwired: 9 in, 1 out]
          }
        }
        n122 = call <vilib>:"Add State(s) to Queue__JKI_lib_State_Machine.vi"("State(s) in (\"\")"=w280) -> ("States Out"=w279:string)  [unwired: 14 in]
      }
      frame "UI: Front Panel State" {
        # "Argument"
        # "Set Front Panel Open or Closed\n(Usage: \"UI: Front Panel State >> Open|Close\")"
        n123 = Unbundle By Name(w287) -> ("Core.Current VI Reference"=w286:refnum<vi>)
        n124 = case shown="\"Minimize\", \"Minimized\"" w285 {
          tunnel: w289 -> [w297 w312 w323 w336 w349]
          tunnel: [w299 w313 w325 w338 w351] -> w288
          tunnel: w286 -> [w298 w310 w324 w337 w350]
          frame "Open", "Standard", Default {
            w292 = T4."Standard" ("State")
            n125 = property class="VI"(reference=w298, error in=w297) -> (reference out=w295:refnum<vi>, error out=w296:errorcluster, "FP.State"=w294:T4)
            n126 = Not Equal?(x=w294, y=w292) -> (x != y?=w293:bool)
            n127 = case shown="True" w293 {
              tunnel: [w303 w305] -> w299
              tunnel: w296 -> [w302 w305]
              tunnel: w295 -> [w301 _]
              tunnel: w292 -> [w300 _]
              frame True {
                n128 = invoke class="VI" method="FP.Open"(reference=w301, error in=w302, "Activate"=TRUE, "State"=w300) -> (error out=w303:errorcluster)  [unwired: 1 in, 4 out]
              }
              frame False {
              }
            }
          }
          frame "Close", "Closed" {
            n129 = property class="VI"(reference=w310, error in=w312) -> (reference out=w309:refnum<vi>, error out=w311:errorcluster, "FP.State"=w307:T4)
            n130 = Not Equal?(x=w307, y=T4."Closed" ("Front Panel Window:State")) -> (x != y?=w306:bool)
            n131 = case shown="True" w306 {
              tunnel: [w314 w317] -> w313
              tunnel: w311 -> [w314 w316]
              tunnel: w309 -> [_ w315]
              frame False {
              }
              frame True {
                n132 = invoke class="VI" method="FP.Close"(reference=w315, error in=w316) -> (error out=w317:errorcluster)  [unwired: 1 in, 2 out]
              }
            }
          }
          frame "Hidden", "Hide" {
            w318 = T4."Hidden" ("State")
            n133 = property class="VI"(reference=w324, error in=w323) -> (reference out=w321:refnum<vi>, error out=w322:errorcluster, "FP.State"=w320:T4)
            n134 = Not Equal?(x=w320, y=w318) -> (x != y?=w319:bool)
            n135 = case shown="True" w319 {
              tunnel: [w329 w330] -> w325
              tunnel: w322 -> [w328 w330]
              tunnel: w321 -> [w327 _]
              tunnel: w318 -> [w326 _]
              frame True {
                n136 = invoke class="VI" method="FP.Open"(reference=w327, error in=w328, "State"=w326) -> (error out=w329:errorcluster)  [unwired: 2 in, 4 out]
              }
              frame False {
              }
            }
          }
          frame "Minimize", "Minimized" {
            w331 = T4."Minimized" ("State")
            n137 = property class="VI"(reference=w337, error in=w336) -> (reference out=w334:refnum<vi>, error out=w335:errorcluster, "FP.State"=w333:T4)
            n138 = Not Equal?(x=w333, y=w331) -> (x != y?=w332:bool)
            n139 = case shown="True" w332 {
              tunnel: [w342 w343] -> w338
              tunnel: w335 -> [w341 w343]
              tunnel: w334 -> [w340 _]
              tunnel: w331 -> [w339 _]
              frame True {
                n140 = invoke class="VI" method="FP.Open"(reference=w340, error in=w341, "State"=w339) -> (error out=w342:errorcluster)  [unwired: 2 in, 4 out]
              }
              frame False {
              }
            }
          }
          frame "Maximize", "Maximized" {
            w344 = T4."Maximized" ("State")
            n141 = property class="VI"(reference=w350, error in=w349) -> (reference out=w347:refnum<vi>, error out=w348:errorcluster, "FP.State"=w346:T4)
            n142 = Not Equal?(x=w346, y=w344) -> (x != y?=w345:bool)
            n143 = case shown="True" w345 {
              tunnel: [w355 w356] -> w351
              tunnel: w348 -> [w354 w356]
              tunnel: w347 -> [w353 _]
              tunnel: w344 -> [w352 _]
              frame True {
                n144 = invoke class="VI" method="FP.Open"(reference=w353, error in=w354, "State"=w352) -> (error out=w355:errorcluster)  [unwired: 2 in, 4 out]
              }
              frame False {
              }
            }
          }
        }
        n145 = call <vilib>:"Add State(s) to Queue__JKI_lib_State_Machine.vi"("State(s) in (\"\")"=w291) -> ("States Out"=w290:string)  [unwired: 14 in]
      }
      frame "CSM: Module List Changed", "UI: Refresh CSM List" {
        n146 = control-ref of="CSM"() -> (w366:refnum<vi>)
        n147 = property on="Property Node" class="CmbBox"(reference=w366) -> (reference out=w358:refnum<vi>, "Value"=w362:string)  [unwired: 1 in, 1 out]
        n148 = call "CSM - List Modules.vi"("Scope (Normal)"="Scope") -> ("error out"=w365:errorcluster, "Module Names"=w360:string[])  [unwired: 9 in]
        n149 = Search 1D Array(1D array=w360, element=w362) -> (index of element=w364:i32)  [unwired: 1 in]
        n150 = Greater Or Equal To 0?(x=w364) -> (x >= 0?=w363:bool)
        n151 = Index Array(array=w360) -> (element=w361:string)  [unwired: 1 in]
        n152 = Select(t=w362, s=w363, f=w361) -> (s? t:f=w359:string)
        n153 = call <vilib>:"Simple Error Handler.vi"("error in (no error)"=w365) -> ()  [unwired: 4 in, 5 out]
        n154 = property on="Property Node" class="CmbBox"(reference=w358, "Strings[]"=w360, "Val(Sgnl)"=w359) -> ()  [unwired: 1 in, 2 out]
      }
      frame "UI: Try to Change Command" {
        n155 = control-ref of="CSM"() -> (w383:refnum<vi>)
        n156 = property on="Property Node" class="CmbBox"(reference=w383) -> (reference out=w373:refnum<vi>, error out=w372:errorcluster, "Strings[]"=w370:string[])  [unwired: 1 in]
        n157 = call "CSM - Convert HexStr to Data.vi"("HEX String"=w382) -> ("Variant"=w380:variant, "error out"=w381:errorcluster)  [unwired: 7 in]
        n158 = Variant To Data(error in=w381, type="", Variant=w380) -> (data=w378:string)  [unwired: 1 out]
        n159 = call "Remove Comments from Single-line.vi"("single-line text"=w378) -> ("single-line text without comments"=w377:string)  [unwired: 2 in]
        n160 = call "Split Single-line Message.vi"("single-line text"=w377) -> ("source/target"=w376:string)  [unwired: 6 in, 3 out]
        n161 = To Lower Case(string=w370) -> (all lower case string=w375:string[])
        n162 = To Lower Case(string=w376) -> (all lower case string=w374:string)
        n163 = Search 1D Array(1D array=w375, element=w374) -> (index of element=w371:i32)  [unwired: 1 in]
        n164 = case shown="Default" w371 {
          selector: w371 -> [_ w388]
          tunnel: w373 -> [_ w391]
          tunnel: w372 -> [_ w390]
          tunnel: w370 -> [_ w389]
          frame -1 {
          }
          frame Default {
            n165 = Index Array(array=w389, index=w388) -> (element=w387:string)
            n166 = property on="Property Node" class="CmbBox"(reference=w391, error in=w390, "Value"=w387) -> ()  [unwired: 2 out]
          }
        }
      }
      frame "UI: Insert LogViewer" {
        # "Replace with your own CSM Module"
        n167 = vi-ref "LogViewer.vi"() -> (w397:refnum<vi>)
        n168 = property class="VI Interface Type 0"(reference=w397) -> (reference out=w401:refnum<vi>, error out=w399:errorcluster, "Path"=w398:path)  [unwired: 1 in]
        n169 = Open VI Reference(type specifier VI Refnum (for type only)=w401, vi path=w398, options=128, error in (no error)=w399) -> (vi reference=w400:refnum<vi>, error out=w396:errorcluster)  [unwired: 2 in]
        n170 = call "Concatenate Submodule Name.vi"("Module Name"="logviewer", "Group Name"=w393) -> ("Submodule Name"=w394:string)  [unwired: 9 in]
        n171 = call-by-ref "Start Asynchronous Call"(reference=w400, error in=w396, "Current Module(\"\" to generate an ID)"=w394) -> (reference out=w395:refnum<vi>, error out=w402:errorcluster)  [unwired: 11 in]
        n172 = invoke on="subpnl" class="SubPnl" method="Insert VI"("VI Ref"=w395) -> ()  [unwired: 3 in, 4 out]
        n173 = Close Reference(reference=w395, error in (no error)=w402) -> ()  [unwired: 1 out]
      }
      frame "UI: Insert History View" {
        n174 = vi-ref "DebugConsole.lvlib:HistoryList.vi"() -> (w413:refnum<vi>)
        n175 = property class="VI Interface Type 0"(reference=w413) -> (reference out=w417:refnum<vi>, error out=w415:errorcluster, "Path"=w414:path)  [unwired: 1 in]
        n176 = Open VI Reference(type specifier VI Refnum (for type only)=w417, vi path=w414, options=128, error in (no error)=w415) -> (vi reference=w416:refnum<vi>, error out=w412:errorcluster)  [unwired: 2 in]
        n177 = call "Concatenate Submodule Name.vi"("Module Name"="historyView", "Group Name"=w409) -> ("Submodule Name"=w410:string)  [unwired: 9 in]
        n178 = call-by-ref "Start Asynchronous Call"(reference=w416, error in=w412, "Current Module(\"\" to generate an ID)"=w410) -> (reference out=w411:refnum<vi>, error out=w418:errorcluster)  [unwired: 11 in]
        n179 = control-ref of="subpnl"() -> (w407:refnum<vi>)
        n180 = invoke on="Invoke Node" class="SubPnl" method="Insert VI"(reference=w407, "VI Ref"=w411) -> ()  [unwired: 2 in, 4 out]
        n181 = Close Reference(reference=w411, error in (no error)=w418) -> ()  [unwired: 1 out]
      }
      frame "UI: Insert Console" {
        n182 = Unbundle By Name(w426) -> ("ConsoleUI"=w425:refnum<vi>[])
        n183 = Index Array(array=w425, index="Console") -> (element=w423:refnum<vi>)
        n184 = control-ref of="subpnl"() -> (w427:refnum<vi>)
        n185 = invoke on="Invoke Node" class="SubPnl" method="Insert VI"(reference=w427, "VI Ref"=w423) -> ()  [unwired: 2 in, 4 out]
      }
      frame "UI: Refresh UI" {
      }
      frame "---------- Macro ----------" {
        # "Do not put any code in this frame.\n(It is a separator no-op. You can make a copy of this frame to create a new Macro frame)"
        n186 = call <vilib>:"Add State(s) to Queue__JKI_lib_State_Machine.vi"("State(s) in (\"\")"=w436) -> ("States Out"=w435:string)  [unwired: 14 in]
      }
      frame "Macro: Initialize" {
        # "Initialization Macro\n(This is called once, when the VI starts)"
        n187 = call <vilib>:"Add State(s) to Queue__JKI_lib_State_Machine.vi"("State(s) in Front (\"\")"="Data: Initialize\nData: Initialize References\nInitialize Core Data\nUI: Initialize\nData: Load Arguments Config File\nUI: Front Panel State >> Open\nAction: Start Message Console\nAction: Start Broadcast Console\nAction: Start Registration Console\nAction: Start Scripts Console\nAction: Start Information Console\nUI: Insert History View\nUI: Insert LogViewer\nUI: Insert Console\nUI: Refresh CSM List\nUI: Refresh UI\nAction: Change Btn States", "State(s) in (\"\")"=w441) -> ("States Out"=w440:string)  [unwired: 13 in]
      }
      frame "Macro: Exit" {
        # "Exit Macro\n(This is called once, when the VI exits)"
        n188 = Concatenate Strings(w442, ".*") -> (w443:string)
        n189 = call "_Broadcast Message.vi"("Module Pattern (support *)"=w443, "Broadcast"=_BroadcastDef."Macro: Exit") -> ("Error out"=w444:errorcluster)  [unwired: 9 in]
        n190 = disable-structure shown="Disabled" {
          disable-tunnel: w444 -> [w455 _]
          disable-tunnel: w442 -> [w453 _]
          frame Disabled {
            n191 = Get Date/Time In Seconds() -> (seconds since 1Jan1904=w454:timestamp)
            n192 = while {
              tunnel: w455 -> [w469]
              tunnel: w453 -> [w468]
              tunnel: w454 -> [w461]
              stop <- w458 stop-if-true
              n193 = call "_Engine.vi"("Enum"=_action."List", "Error in"=w469) -> ("Array"=w466:string[])  [unwired: 7 in, 2 out]
              n194 = Get Date/Time In Seconds() -> (seconds since 1Jan1904=w462:timestamp)
              n195 = Search 1D Array(1D array=w466, element=w468) -> (index of element=w467:i32)  [unwired: 1 in]
              n196 = Subtract(x=w462, y=w461) -> (x-y=w460:dbl)
              n197 = Delete From Array(array=w466, index=w467) -> (array with subset deleted=w465:string[])  [unwired: 1 in, 1 out]
              n198 = Greater?(x=w460, y=5.0) -> (0:w456:bool)
              n199 = Empty Array?(array=w465) -> (empty?=w457:bool)
              n200 = Wait (ms)(milliseconds to wait=u32 10) -> ()  [unwired: 1 out]
              n201 = Or(x=w457, y=w456) -> (x .or. y?=w458:bool)
            }
          }
          frame Enabled {
          }
        }
        n202 = call <vilib>:"Add State(s) to Queue__JKI_lib_State_Machine.vi"("State(s) at Back (\"\")"="Data: Save Arguments Config File\nData: Cleanup\nExit") -> ("States Out"=w447:string)  [unwired: 14 in]
        n203 = call <vilib>:"Add State(s) to Queue__JKI_lib_State_Machine.vi"("State(s) in Front (\"\")"=w447, "State(s) in (\"\")"=w452) -> ("States Out"=w451:string)  [unwired: 13 in]
      }
      frame "---------- Action ----------" {
        # "Template Separator\n(You can make a copy of, or modify, this frame)"
        n204 = call <vilib>:"Add State(s) to Queue__JKI_lib_State_Machine.vi"("State(s) in (\"\")"=w473) -> ("States Out"=w472:string)  [unwired: 14 in]
      }
      frame "Action: Change Btn States" {
        n205 = local read "CSM"() -> (w477:string)
        n206 = case shown="Default" w477 {
          selector: w477 -> [_ w481]
          tunnel: w476 -> [_ w494]
          frame "" {
          }
          frame Default {
            n207 = call "CSM - Module VI Reference.vi"("Response Timeout (-2 Using Global Settings)"=1000 ("Response Timeout(5000 ms)"), "Current Module (\"\" to Generate an ID)"=w494, "CSM Name"=w481) -> ("error out"=w491:errorcluster, "CSM Module VIRef"=w492:refnum<vi>)  [unwired: 7 in]
            n208 = property class="VI"(reference=w492, error in=w491) -> (reference out=w485:refnum<vi>, "IsInPackedLibrary"=→"inlvlibp":bool, "Diagram"=w484:refnum<vi>)  [unwired: 1 out]
            n209 = Close Reference(reference=w484) -> (error out=w483:errorcluster)  [unwired: 1 in]
            n210 = call <vilib>:"Clear Errors.vi"("error in (no error)"=w483) -> ("error out"=w482:errorcluster)  [unwired: 5 in, 1 out]
            n211 = Close Reference(reference=w485, error in (no error)=w482) -> ()  [unwired: 1 out]
            n212 = Not A Number/Path/Refnum?(number/path/refnum=w484) -> (NaN/Path/Refnum?=w488:bool)
            n213 = Select(t=2, s=w488, f=0) -> (s? t:f=w489:i32)
            n214 = property on="Toolbar.Open BD" class="Bool"("DisabledEnum"=w489) -> ()  [unwired: 2 in, 2 out]
          }
        }
        n215 = local read "CSM"() -> (w475:string)
        n216 = call "_Broadcast Message.vi"("Argument(\"\")"=w475, "Broadcast"=_BroadcastDef."CSM: Module Selected") -> ()  [unwired: 9 in, 1 out]
      }
      frame "No Peroidic Log over 1s" {
        n217 = call "CSM - Generate User Global Log.vi"("Place (\"\" to Use VI's Name)"=w495, "Log"="No Peroidic Log over 1s.") -> ()  [unwired: 9 in, 1 out]
      }
      frame "Action: Start Message Console" {
        n218 = in-place {
          in-place-border: w500 -> [w506]
          # "Replace with your own CSM Module"
          n219 = in-place-cluster #1(w502) -> ("ConsoleUI"=w510:refnum<vi>[])
          n220 = vi-ref "Message Console.vi"() -> (w513:refnum<vi>)
          n221 = property class="VI Interface Type 0"(reference=w513) -> (reference out=w517:refnum<vi>, error out=w515:errorcluster, "Path"=w514:path)  [unwired: 1 in]
          n222 = Open VI Reference(type specifier VI Refnum (for type only)=w517, vi path=w514, options=128, error in (no error)=w515) -> (vi reference=w516:refnum<vi>, error out=w512:errorcluster)  [unwired: 2 in]
          n223 = call "Concatenate Submodule Name.vi"("Module Name"="MsgConsole", "Group Name"=w506) -> ("Submodule Name"=w505:string)  [unwired: 9 in]
          n224 = call-by-ref "Start Asynchronous Call"(reference=w516, error in=w512, "Name"=w505) -> (reference out=w508:refnum<vi>, error out=w518:errorcluster)  [unwired: 11 in]
          n225 = Close Reference(reference=w508, error in (no error)=w518) -> ()  [unwired: 1 out]
          n226 = Build Array (concatenate)(w510, w508) -> (w509:refnum<vi>[])
          n227 = in-place-cluster #1("ConsoleUI"=w509) -> (w501:T9)
        }
      }
      frame "Action: Start Broadcast Console" {
        n228 = in-place {
          in-place-border: w519 -> [w525]
          # "Replace with your own CSM Module"
          n229 = in-place-cluster #2(w521) -> ("ConsoleUI"=w529:refnum<vi>[])
          n230 = vi-ref "Broadcast Console.vi"() -> (w532:refnum<vi>)
          n231 = property class="VI Interface Type 0"(reference=w532) -> (reference out=w536:refnum<vi>, error out=w534:errorcluster, "Path"=w533:path)  [unwired: 1 in]
          n232 = Open VI Reference(type specifier VI Refnum (for type only)=w536, vi path=w533, options=128, error in (no error)=w534) -> (vi reference=w535:refnum<vi>, error out=w531:errorcluster)  [unwired: 2 in]
          n233 = call "Concatenate Submodule Name.vi"("Module Name"="BroadcastConsole", "Group Name"=w525) -> ("Submodule Name"=w524:string)  [unwired: 9 in]
          n234 = call-by-ref "Start Asynchronous Call"(reference=w535, error in=w531, "name"=w524) -> (reference out=w527:refnum<vi>, error out=w537:errorcluster)  [unwired: 11 in]
          n235 = Close Reference(reference=w527, error in (no error)=w537) -> ()  [unwired: 1 out]
          n236 = Build Array (concatenate)(w529, w527) -> (w528:refnum<vi>[])
          n237 = in-place-cluster #2("ConsoleUI"=w528) -> (w520:T9)
        }
      }
      frame "Action: Start Registration Console" {
        n238 = in-place {
          in-place-border: w538 -> [w544]
          # "Replace with your own CSM Module"
          n239 = in-place-cluster #3(w540) -> ("ConsoleUI"=w549:refnum<vi>[])
          n240 = vi-ref "Registration Console.vi"() -> (w546:refnum<vi>)
          n241 = property class="VI Interface Type 0"(reference=w546) -> (reference out=w555:refnum<vi>, error out=w553:errorcluster, "Path"=w552:path)  [unwired: 1 in]
          n242 = Open VI Reference(type specifier VI Refnum (for type only)=w555, vi path=w552, options=128, error in (no error)=w553) -> (vi reference=w554:refnum<vi>, error out=w551:errorcluster)  [unwired: 2 in]
          n243 = call "Concatenate Submodule Name.vi"("Module Name"="RegConsole", "Group Name"=w544) -> ("Submodule Name"=w545:string)  [unwired: 9 in]
          n244 = call-by-ref "Start Asynchronous Call"(reference=w554, error in=w551, "name"=w545) -> (reference out=w547:refnum<vi>, error out=w556:errorcluster)  [unwired: 11 in]
          n245 = Close Reference(reference=w547, error in (no error)=w556) -> ()  [unwired: 1 out]
          n246 = Build Array (concatenate)(w549, w547) -> (w548:refnum<vi>[])
          n247 = in-place-cluster #3("ConsoleUI"=w548) -> (w539:T9)
        }
      }
      frame "Action: Start Scripts Console" {
        n248 = in-place {
          in-place-border: w557 -> [w563]
          # "Replace with your own CSM Module"
          n249 = in-place-cluster #4(w559) -> ("ConsoleUI"=w568:refnum<vi>[])
          n250 = vi-ref "DebugConsole.lvlib:Script-Window.vi"() -> (w565:refnum<vi>)
          n251 = property class="VI Interface Type 0"(reference=w565) -> (reference out=w574:refnum<vi>, error out=w572:errorcluster, "Path"=w571:path)  [unwired: 1 in]
          n252 = Open VI Reference(type specifier VI Refnum (for type only)=w574, vi path=w571, options=128, error in (no error)=w572) -> (vi reference=w573:refnum<vi>, error out=w570:errorcluster)  [unwired: 2 in]
          n253 = call "Concatenate Submodule Name.vi"("Module Name"="ScriptConsole", "Group Name"=w563) -> ("Submodule Name"=w564:string)  [unwired: 9 in]
          n254 = call-by-ref "Start Asynchronous Call"(reference=w573, error in=w570, "name"=w564) -> (reference out=w566:refnum<vi>, error out=w575:errorcluster)  [unwired: 11 in]
          n255 = Close Reference(reference=w566, error in (no error)=w575) -> ()  [unwired: 1 out]
          n256 = Build Array (concatenate)(w568, w566) -> (w567:refnum<vi>[])
          n257 = in-place-cluster #4("ConsoleUI"=w567) -> (w558:T9)
        }
      }
      frame "Action: Start Information Console" {
        n258 = in-place {
          in-place-border: w576 -> [w582]
          n259 = in-place-cluster #5(w578) -> ("ConsoleUI"=w587:refnum<vi>[])
          n260 = vi-ref "DebugConsole.lvlib:Module Information.vi"() -> (w584:refnum<vi>)
          n261 = property class="VI Interface Type 0"(reference=w584) -> (reference out=w593:refnum<vi>, error out=w591:errorcluster, "Path"=w590:path)  [unwired: 1 in]
          n262 = Open VI Reference(type specifier VI Refnum (for type only)=w593, vi path=w590, options=128, error in (no error)=w591) -> (vi reference=w592:refnum<vi>, error out=w589:errorcluster)  [unwired: 2 in]
          n263 = call "Concatenate Submodule Name.vi"("Module Name"="ModuleInfo", "Group Name"=w582) -> ("Submodule Name"=w583:string)  [unwired: 9 in]
          n264 = call-by-ref "Start Asynchronous Call"(reference=w592, error in=w589, "name"=w583) -> (reference out=w585:refnum<vi>, error out=w594:errorcluster)  [unwired: 11 in]
          n265 = Close Reference(reference=w585, error in (no error)=w594) -> ()  [unwired: 1 out]
          n266 = Build Array (concatenate)(w587, w585) -> (w586:refnum<vi>[])
          n267 = in-place-cluster #5("ConsoleUI"=w586) -> (w577:T9)
        }
      }
    }
  }
  n268 = disable-structure shown="Disabled" {
    frame Disabled {
      n269 = case shown="\"Module Created\", \"Module Destroyed\"" {
        selector: _ -> [_ _]
        tunnel: _ -> [_ w596]
        frame "User Log", Default {
        }
        frame "Module Created", "Module Destroyed" {
          n270 = Generate User Event(user event=w596, event data cluster="UI: Refresh CSM List" ("State(s) in Front (\"\")")) -> ()  [unwired: 2 in, 2 out]
        }
      }
    }
    frame Enabled {
    }
  }
  n271 = control-ref of="Current VI Reference"() -> (w3:refnum<vi>)
  n272 = call "Close FP if in LabVIEW Dir.vi"("VI Refnum"=w3, "Error in"=w2) -> ("Error out"=w4:errorcluster)  [unwired: 9 in]
  n273 = call <vilib>:"Clear Errors.vi"("error in (no error)"=w4) -> ()  [unwired: 5 in, 2 out]
